vi "Data filter.vi"(11 "Array":dbl[](array[numeric])) -> (3 "True":bool)   [LabVIEW 2026]
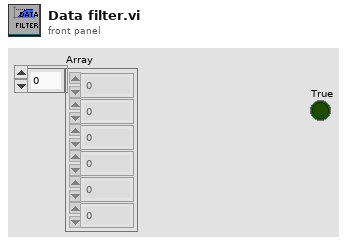
[diagram p1: front panel]
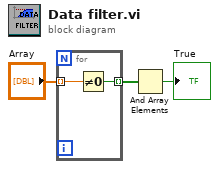
[diagram p0: block diagram]
diagram:
  n1 = for {
    tunnel: "Array" -> [w5] mode=indexing
    tunnel: [w4] -> w2 mode=indexing
    n2 = Not Equal To 0?(x=w5) -> (x != 0?=w4:bool)
  }
  n3 = And Array Elements(Boolean array=w2) -> (logical AND=→"True":bool)
